vi "2_Power_Transmission_Line_Fault_Classification(Inference).vi"() -> ()   [LabVIEW 2020]
uses:
  <vilib>/Ngene/Deep Learning Toolkit/Toolkit/NN_Network/Controls/NN_Save_Before_Destroy_Options.ctl
  <vilib>/Ngene/Deep Learning Toolkit/Toolkit/NN_Network/API/NN_Set_Input/1D/NN_Set_Input(1D_SGL_idx).vi
  <vilib>/Ngene/Deep Learning Toolkit/Toolkit/Deep_Learning_Toolkit_by_Ngene.lvlib
  <vilib>/measure/NI_MABase.lvlib
panel:
  in  "Position":dbl(slide)=0.8028391167192429 scale=0.0..1.0
  in  "Fault Generation":T1(tab)=enum."Transient"
  in  "scale":sgl(slide)=0.65 scale=0.5..0.65
  in  "Duration(#s)":i32(slide)=496 scale=300.0..600.0
  in  "scale":sgl(slide)=1.5083333 scale=1.4..1.6
  in  "Duration(#s)":i32(slide)=351 scale=300.0..600.0
  in  "Duration(#s)":i32(slide)=231 scale=200.0..600.0
  in  "Tau":dbl(slide)=150.0 scale=130.0..150.0
  in  "Frequency":dbl(slide)=1000.0 scale=500.0..1500.0
  in  "Amplitude":dbl(slide)=126.5625 scale=100.0..150.0
  in  "Offset":sgl(slide)=138.54167 scale=50.0..150.0
  in  "Duration(#s)":i32(slide)=262 scale=200.0..600.0
  out "Predicted Class":string="Transient"
  out "Class Labels":string[](array[string])=["DC Offset", "Interruption", "Normal", "Sag", "Swell", "Transient"]
  out "Generated WaveForm":waveform(sgl)(graph)={"t0"=timestamp(0 s since 1904-01-01), "dt"=1.0, "Y"=array[2000 elements]}
  in  "Weight File Path":path=path "D:/Ngene/GitHub/deepltk_examples/2_Waveform_Processing/23_Power_Transmission_Line_Fault_Classification/working/Fault_Classifier/Fault_Classifier_weights_25_06_11__13_19_35.bin"
  in  "Configuration File Path":path=path "D:/Ngene/GitHub/deepltk_examples/2_Waveform_Processing/23_Power_Transmission_Line_Fault_Classification/working/Fault_Classifier/Fault_Classifier_net_cfg_25_06_11__13_19_35.cfg"
  out "Class Probabilities":sgl[](array[slide])=[0.0010221456, 7.1583037e-07, 7.443848e-05, 0.02422408, 0.014738527, 0.9599401] scale=0.0..1.0
  in  "Stop":bool
  # "Overview: Demonstrates the usage of DeepLTK for loading the model pretrained for Power Line Fault Classification and running for inference.\nRequirements: DeepLTK - Deep Learning Toolkit for LabVIEW (https://www.ngene.co/deep-learning-toolkit-for-labview)\nInstructions:\n1. Provide Network Configuration File Path and Weight File Path generated from training example.\n2. Run the VI\n3. Choose type of the fault, change the parameters and observe the predicted type of the fault.\n4. Press the Stop button to stop the VI.\n\nMore Examples:  https://github.com/ngenehub/deepltk_examples"
  # "Power Transmission Line Fault Classification - Inference"
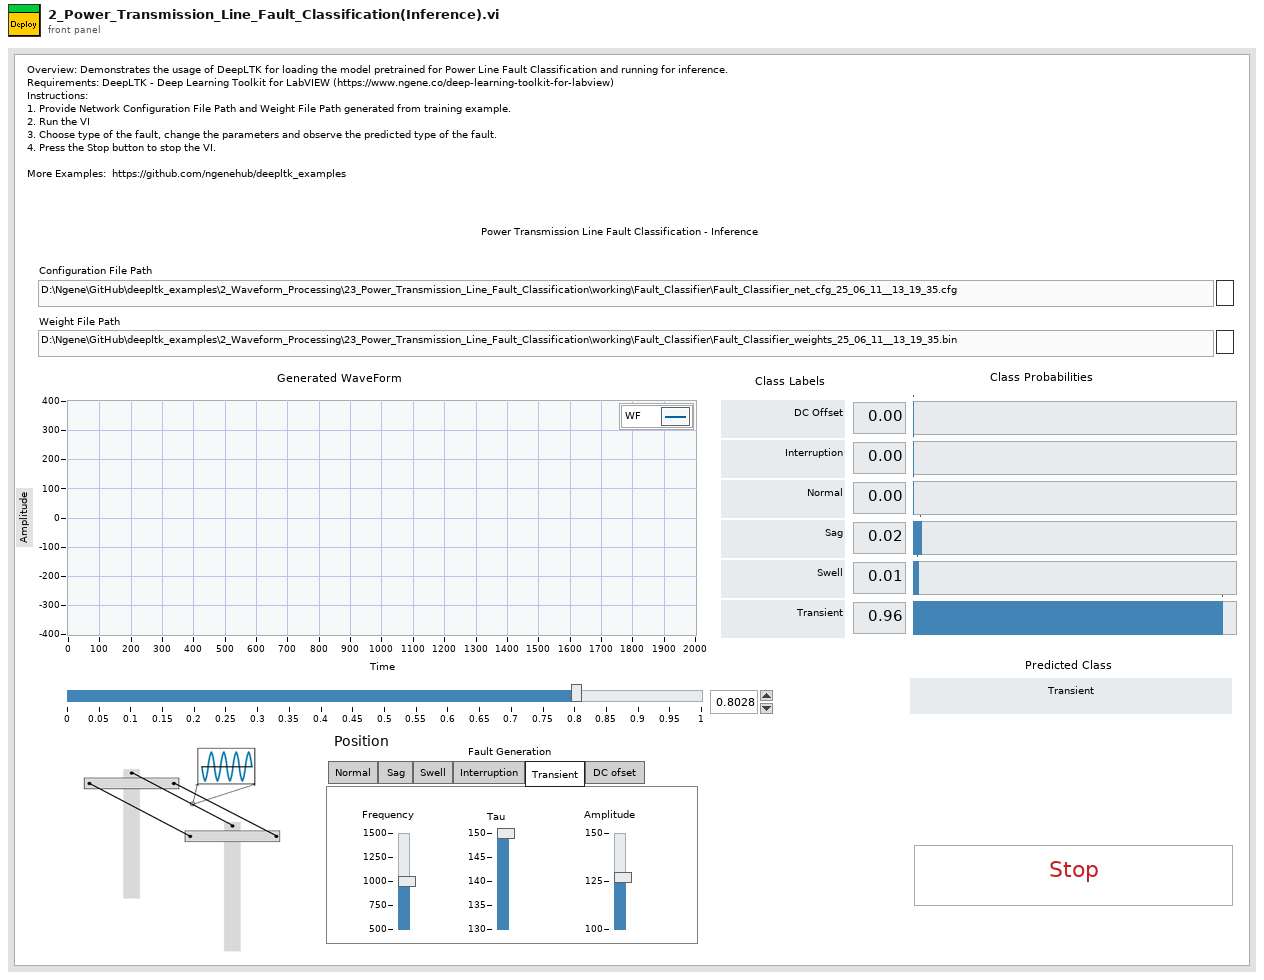
[diagram p1: front panel]
types:
  T1 = enum32{"Normal", "Sag ", "Swell", "Interruption", "Transient", "DC ofset "}
  T2 = typedef "Deep_Learning_Toolkit_by_Ngene.lvlib/NN_Save_Before_Destroy_Options.ctl" = cluster{"CFG?":bool, "Weights?":bool, "Render?":bool}
  T3 = typedef "Deep_Learning_Toolkit_by_Ngene.lvlib/NN_Config_Params.ctl" = cluster{"Name":string, "mBatch":i32, "NN_Train_Params":T4, "LR_Decay_Policy":T7, "Labels":string[], "Loss":T9, "Max_WS_Size(B)":i64, "DryRun?":bool}
  T4 = typedef "Deep_Learning_Toolkit_by_Ngene.lvlib/NN_Train_Params.ctl" = cluster{"Optimizer":T5, "Beta_1":sgl, "Beta_2":sgl, "Weight Decay(L1)":sgl, "Weight Decay(L2)":sgl, "Data_Sampling":T6}
  T5 = typedef "Deep_Learning_Toolkit_by_Ngene.lvlib/NN_Train_Optimizer.ctl" = enum16{"SGD", "Adam", "Adagrad", "Adadelta", "RMSProp", "Nesterov"}
  T6 = typedef "Deep_Learning_Toolkit_by_Ngene.lvlib/NN_Train_Data_Sampling.ctl" = enum16{"Random", "Sequential"}
  T7 = typedef "Deep_Learning_Toolkit_by_Ngene.lvlib/NN_LR_Policy_Cfg.ctl" = cluster{"Policy_Type":T8, "LR0":dbl, "k":sgl, "WarmUp_Policy":enum16{"Step", "Ramp"}, "WarmUp_Iter":i32, "WarmUp_Ratio":sgl}
  T8 = typedef "Deep_Learning_Toolkit_by_Ngene.lvlib/NN_LR_Policy_Type.ctl" = enum16{"Manual", "Step", "Exp", "1/t"}
  T9 = typedef "Deep_Learning_Toolkit_by_Ngene.lvlib/NN_Loss_Config_Params.ctl" = cluster{"Loss_Type":T10, "Loss_Conf_Params":variant}
  T10 = typedef "Deep_Learning_Toolkit_by_Ngene.lvlib/NN_Loss_Type.ctl" = enum16{"None", "MSE", "CrossEntropy", "YOLO_v2", "YOLO_v4"}
  T11 = typedef "Deep_Learning_Toolkit_by_Ngene.lvlib/NN_Layer_Config_Params.ctl" = cluster{"Layer_Type":T12, "Layer_Conf_Params":variant, "Input Layers":string[]}
  T12 = typedef "Deep_Learning_Toolkit_by_Ngene.lvlib/NN_Layer_Type.ctl" = enum16{"Input1D", "Input3D", "Conv1D", "Conv2D", "Conv2D_Adv", "MaxPool", "AvgPool", "UpSample", "DropOut3D", "ShortCut", "Concat", "SoftMax3D", "FC", "DropOut", "Softmax", "Flatten", "YOLO_v2", "YOLO_v4", "Activation", "BatchNormalization", "LayerNormalization", "Scale", "Unsupported"}
  T13 = typedef "Deep_Learning_Toolkit_by_Ngene.lvlib/NN.ctl" = cluster{"Name":string, "No of Layers":i32, "mBatch":i32, "Layers":T14[], "Dimty":T15, "Dims_In":T16, "Dims_Out":T16, "Working_Dir":path, "Train?":bool, "Train_Params":T4, "LR_Update_Policy":T7, "Session Data":T17, "Ground_truth":T18, "NNg_hdls":T19, "NN_Device":T20, "GPU Id":i32, "Labels":string[], "Loss_Type":T10, "Loss_Cfg_Prms":variant, "NNG_WS":T21, "DryRun?":bool}
  T14 = typedef "Deep_Learning_Toolkit_by_Ngene.lvlib/NN_Layer_ref.ctl" = refnum<file>
  T15 = typedef "Deep_Learning_Toolkit_by_Ngene.lvlib/NN_In_Out_Dim-ty.ctl" = enum8{"In1D_Out1D", "In3D_Out1D", "In3D_Out3D", "In3D_OutBBox"}
  T16 = typedef "Deep_Learning_Toolkit_by_Ngene.lvlib/NN_Dims(C,H,W).ctl" = cluster{"C":i32, "H":i32, "W":i32}
  T17 = typedef "Deep_Learning_Toolkit_by_Ngene.lvlib/NN_Train_Session_Data.ctl" = cluster{"Epochs":sgl, "Tot_Iter":i32, "LR":sgl, "LR_iter":i32}
  T18 = typedef "Deep_Learning_Toolkit_by_Ngene.lvlib/NN_Ground_truth.ctl" = cluster{"Y":variant}
  T19 = typedef "Deep_Learning_Toolkit_by_Ngene.lvlib/nng_cuda_handles.ctl" = cluster{"cudnn":u64, "cublas":u64, "stream":u64, "curand":u64}
  T20 = typedef "Deep_Learning_Toolkit_by_Ngene.lvlib/NN_Device.ctl" = enum16{"CPU", "GPU"}
  T21 = typedef "Deep_Learning_Toolkit_by_Ngene.lvlib/NNG_WS.ctl" = cluster{"NNG_WS_Mem":T22, "Max_WS_Size":i64}
  T22 = typedef "Deep_Learning_Toolkit_by_Ngene.lvlib/NNg_WS_Mem_DVR.ctl" = refnum<data-value>
  T23 = typedef "Deep_Learning_Toolkit_by_Ngene.lvlib/NN_Layer.ctl" = cluster{"Name":string, "Layer_Data":T24, "Layer_Type":T12, "Dims_In":T16, "Layers_In":T14[], "Dims_Out":T16, "Layers_Out":T14[], "Metrics":T25, "GPU_Data":T26, "mBatch":i32, "NN_Device":T20, "NNg_hdls":T19, "Train?":bool, "Dimty":T27, "RecptField":T28, "Idx":i32}
  T24 = typedef "Deep_Learning_Toolkit_by_Ngene.lvlib/NN_Layer_Data_Refnum.ctl" = refnum<file>
  T25 = typedef "Deep_Learning_Toolkit_by_Ngene.lvlib/NN_Layer_Metrics.ctl" = cluster{"Data":dbl, "Params":dbl, "Ops":dbl}
  T26 = typedef "Deep_Learning_Toolkit_by_Ngene.lvlib/NNg_Layer_Data_Refnum.ctl" = refnum<file>
  T27 = typedef "Deep_Learning_Toolkit_by_Ngene.lvlib/NN_Layer_Dimty.ctl" = enum16{"1D", "3D"}
  T28 = typedef "Deep_Learning_Toolkit_by_Ngene.lvlib/NN_Layer_RF_State.ctl" = cluster{"Dims":T29, "J":T29}
  T29 = typedef "Deep_Learning_Toolkit_by_Ngene.lvlib/NN_Dims(V,H).ctl" = cluster{"V":i32, "H":i32}
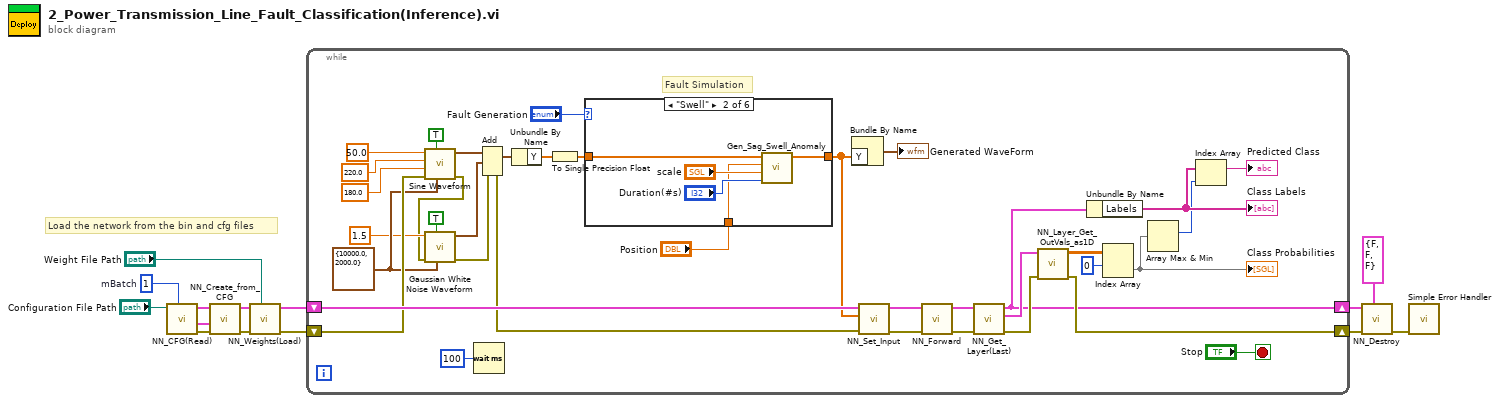
[diagram p0: block diagram]
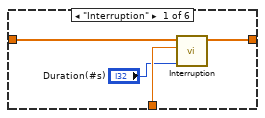
[diagram p2: hidden frame]
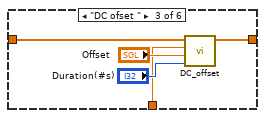
[diagram p3: hidden frame]
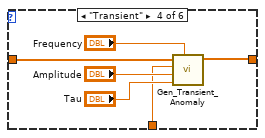
[diagram p4: hidden frame]
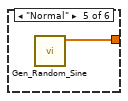
[diagram p5: hidden frame]
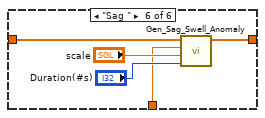
[diagram p6: hidden frame]
diagram:
  w1 = 1  # mBatch
  # "Load the network from the bin and cfg files"
  n1 = call <vilib>:"NN_CFG(Read).vi"("mBatch"=w1, "CFG file path"="Configuration File Path") -> ("error out"=w8:errorcluster, "Net_Cfg"=w9:T3, "Layer_Cfg"=w7:T11[])  [unwired: 7 in]
  n2 = call <vilib>:"NN_Create_from_CFG.vi"("error in (no error)"=w8, "Net_Cfg"=w9, "Layer_Cfg"=w7) -> ("error out"=w11:errorcluster, "NN out"=w6:T13)  [unwired: 7 in]
  n3 = call <vilib>:"NN_Weights(Load).vi"("Weight File Path"="Weight File Path", "error in (no error)"=w11, "NN in"=w6) -> ("error out"=w5:errorcluster, "NN out"=w4:T13)  [unwired: 7 in]
  n4 = while {
    shift-right: [w51] -> w14
    shift-left: w5 -> [w24]
    shift-right: [w40] -> w13
    shift-left: w4 -> [w41]
    stop <- "Stop" stop-if-true
    w22 = cluster{"Fs":dbl, "#s":dbl} {"Fs"=10000.0, "#s"=2000.0} ("sampling info")
    # "Fault Simulation"
    n5 = call <vilib>:"Sine Waveform.vi"("sampling info"=w22, "reset signal"=TRUE, "error in (no error)"=w24, "phase"=180.0, "amplitude"=220.0, "frequency"=50.0) -> ("error out"=w16:errorcluster, "signal out"=w33:waveform(dbl))  [unwired: 4 in]
    n6 = call <vilib>:"Gaussian White Noise Waveform.vi"("sampling info"=w22, "reset signal"=TRUE, "error in (no error)"=w16, "standard deviation"=sgl 1.5 ("Noise Standart Deviation")) -> ("error out"=w15:errorcluster, "signal out"=w17:waveform(dbl))  [unwired: 6 in]
    n7 = Wait (ms)(milliseconds to wait=u32 100) -> ()  [unwired: 1 out]
    n8 = Add(1:w17, 2:w33, 4:w15) -> (0:w20:waveform(dbl), 3:w18:errorcluster)
    n9 = Unbundle By Name(w20) -> ("Y"=w32:dbl[])
    n10 = To Single Precision Float(number=w32) -> (single precision float=w28:sgl[])
    n11 = case shown="\"Swell\"" "Fault Generation" {
      tunnel: [w54 w57 w62 w70 w72 w74] -> w30
      tunnel: w28 -> [w55 w60 w65 w71 _ w77]
      tunnel: "Position" -> [w53 w56 w61 w66 _ w73]
      frame "Interruption" {
        n12 = call "Interruption.vi"("Duration"="Duration(#s)", "Position"=w53, "Sine"=w55) -> ("Sine+Anomaly"=w54:sgl[])  [unwired: 8 in]
      }
      frame "Swell" {
        n13 = call "Gen_Sag_Swell_Anomaly.vi"("Duration"="Duration(#s)", "Amplitude"="scale", "Position"=w56, "Sine"=w60) -> ("Sine+Anomaly"=w57:sgl[])  [unwired: 7 in]
      }
      frame "DC ofset " {
        n14 = call "DC_offset.vi"("Duration"="Duration(#s)", "Ampltude"="Offset", "Position"=w61, "Sine"=w65) -> ("Sine+Anomaly"=w62:sgl[])  [unwired: 7 in]
      }
      frame "Transient" {
        n15 = call "Gen_Transient_Anomaly.vi"("Frequency"="Frequency", "Tau"="Tau", "Amplitude"="Amplitude", "Position"=w66, "Sine"=w71) -> ("Sine+Anomaly"=w70:sgl[])  [unwired: 6 in]
      }
      frame "Normal" {
        n16 = call "Gen_Random_Sine.vi"() -> ("data"=w72:sgl[])  [unwired: 11 in]
      }
      frame "Sag " {
        n17 = call "Gen_Sag_Swell_Anomaly.vi"("Duration"="Duration(#s)", "Amplitude"="scale", "Position"=w73, "Sine"=w77) -> ("Sine+Anomaly"=w74:sgl[])  [unwired: 7 in]
      }
    }
    n18 = Bundle By Name("Y"=w30) -> (→"Generated WaveForm":waveform(sgl))  [unwired: 1 in]
    n19 = call-poly <vilib>:"NN_Set_Input.vi"("error in (no error)"=w18, "Data_In(1D_SGL)"=w30, "NN In"=w41) -> ("error out"=w50:errorcluster, "NN Out"=w47:T13)  [unwired: 7 in]
    n20 = call <vilib>:"NN_Forward.vi"("error in (no error)"=w50, "NN in"=w47) -> ("error out"=w49:errorcluster, "NN out"=w48:T13)  [unwired: 6 in, 2 out]
    n21 = call <vilib>:"NN_Get_Layer(Last).vi"("error in (no error)"=w49, "NN in"=w48) -> ("error out"=w46:errorcluster, "Last_Layer"=w45:T23, "NN out"=w40:T13)  [unwired: 6 in, 1 out]
    n22 = call <vilib>:"NN_Layer_Get_OutVals_as1D.vi"("error in (no error)"=w46, "Layer"=w45) -> ("error out"=w51:errorcluster, "Out(as1D)"=w44:sgl[][])  [unwired: 8 in]
    n23 = Unbundle By Name(w40) -> ("Labels"=w37:string[])
    "Class Labels" <- w37
    n24 = Index Array(array=w44, index (row)=0) -> (element=w38:sgl[])  [unwired: 1 in]
    "Class Probabilities" <- w38
    n25 = Array Max & Min(array=w38) -> (max index (indices)=w36:i32)  [unwired: 3 out]
    n26 = Index Array(array=w37, index=w36) -> (element=→"Predicted Class":string)
  }
  n27 = call <vilib>:"NN_Destroy.vi"("Save (T, T, T)"=T2 {"CFG?"=FALSE, "Weights?"=FALSE, "Render?"=FALSE}, "error in (no error)"=w14, "NN in"=w13) -> ("error out"=w2:errorcluster)  [unwired: 7 in, 1 out]
  n28 = call <vilib>:"Simple Error Handler.vi"("error in (no error)"=w2) -> ()  [unwired: 4 in, 5 out]
